vi "LEDComms.vi"() -> (0 "error out":errorcluster)   [LabVIEW 2017]
uses:
  Implements/TypeDefs/IntakeState.ctl
  <vilib>/Rock Robotics/SystemInterfaces/i2clib/i2c_bus.ctl
  Global_Var-RefNum/LEDData.vi
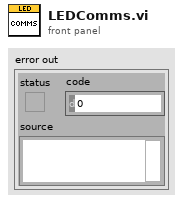
[diagram p1: front panel]
types:
  T1 = typedef "ArmTargetPosition.ctl" = enum16{"Hold", "Switch", "Scale Low", "Scale High", "Climb", "Back Place"}
  T2 = typedef "WPI_DriverStationRobotMode2.ctl" = enum16{"Autonomous Disabled", "Autonomous Enabled", "Teleop Disabled", "Teleop Enabled", "Disconnected", "Finish", "Test Disabled", "Test Enabled", "Emergency Stopped"}
  T3 = typedef "IntakeState.ctl" = enum16{"Stop", "Forward", "Reverse", "Forward Open"}
  T4 = typedef "LEDAutoMode.ctl" = enum16{"Auto Left Switch", "Auto Left Scale", "Auto Center Switch", "Auto Center Scale", "Auto Right Switch", "Auto Right Scale", "Auto Line"}
  T5 = typedef "WPI_I2CDevRef.ctl" = cluster{"DevStatus":errorcluster, "Device Address":u8, "Handle":i32, "I2C Bus":T6}
  T6 = typedef "i2c_bus.ctl" = enum16{"I2C On-Board", "I2C MXP", "Invalid"}
  T7 = typedef "WPI_DriverStationAllianceInfo.ctl" = enum16{"Red", "Blue", "Invalid"}
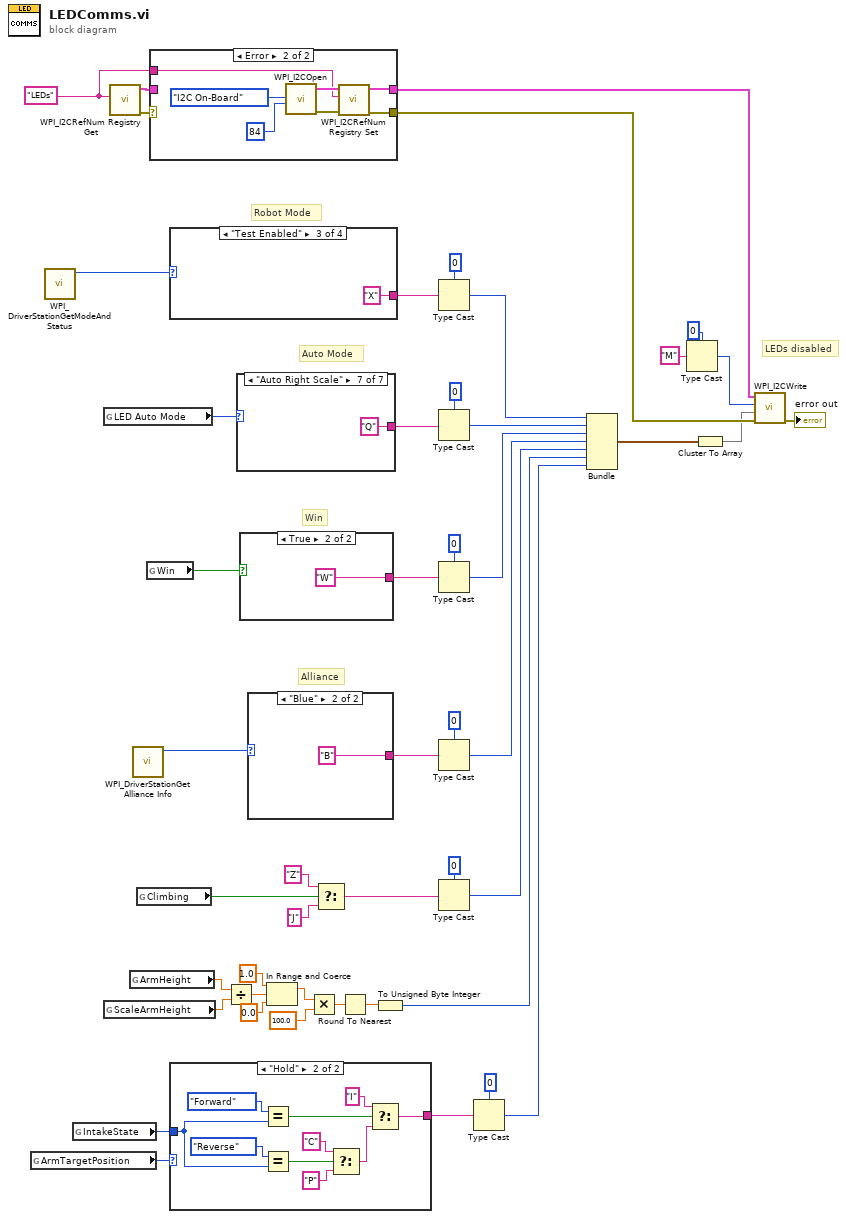
[diagram p0: block diagram]
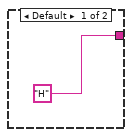
[diagram p2: hidden frame]
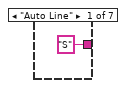
[diagram p4: hidden frame]
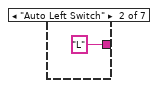
[diagram p5: hidden frame]
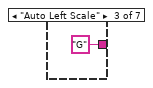
[diagram p6: hidden frame]
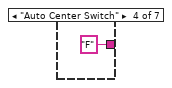
[diagram p7: hidden frame]
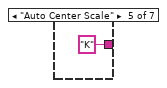
[diagram p8: hidden frame]
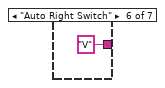
[diagram p9: hidden frame]
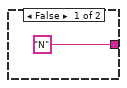
[diagram p10: hidden frame]
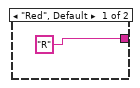
[diagram p11: hidden frame]
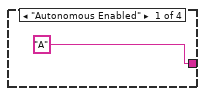
[diagram p12: hidden frame]
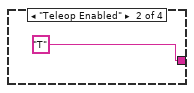
[diagram p13: hidden frame]
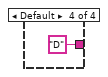
[diagram p14: hidden frame]
diagram:
  w23 = "LEDs" ("refnum name")
  # "LEDs disabled"
  # "Alliance"
  # "Win"
  # "Robot Mode"
  # "Auto Mode"
  n1 = global read "LEDData.vi" "ArmTargetPosition"() -> (w4:T1)
  n2 = call <vilib>:"WPI_DriverStationGetModeAndStatus.vi"() -> ("Robot Mode"=w30:T2)  [unwired: 10 in, 1 out]
  n3 = global read "LEDData.vi" "IntakeState"() -> (w2:T3)
  n4 = global read "LEDData.vi" "LED Auto Mode"() -> (w20:T4)
  n5 = global read "LEDData.vi" "ScaleArmHeight"() -> (w13:dbl)
  n6 = call <vilib>:"WPI_I2CRefNum Registry Get.vi"("refnum name"=w23) -> ("error out"=w21:errorcluster, "I2CDevRef"=w22:T5)  [unwired: 9 in]
  n7 = global read "LEDData.vi" "ArmHeight"() -> (w14:dbl)
  n8 = call <vilib>:"WPI_DriverStationGet Alliance Info.vi"() -> ("Alliance"=w39:T7)  [unwired: 6 in, 5 out]
  n9 = global read "LEDData.vi" "Climbing"() -> (w16:bool)
  n10 = global read "LEDData.vi" "Win"() -> (w19:bool)
  n11 = case shown="Error" w21 {
    selector: w21 -> [w50 _]
    tunnel: [w50 w52] -> w48
    tunnel: [w49 w53] -> w47
    tunnel: w22 -> [w49 _]
    tunnel: w23 -> [_ w51]
    frame No Error {
    }
    frame Error {
      n12 = call <vilib>:"WPI_I2COpen.vi"("Device Address"=u8 84, "I2C Bus"=i2c_bus."I2C On-Board") -> ("error out"=w55:errorcluster, "I2CDevRef"=w54:T5)  [unwired: 8 in]
      n13 = call <vilib>:"WPI_I2CRefNum Registry Set.vi"("error in (no error)"=w55, "refnum name"=w51, "I2CDevRef"=w54) -> ("error out"=w52:errorcluster, "I2CDevRef"=w53:T5)  [unwired: 7 in]
    }
  }
  n14 = case shown="\"Test Enabled\"" w30 {
    tunnel: ["A" "T" "X" "D"] -> w42
    frame "Autonomous Enabled" {
    }
    frame "Teleop Enabled" {
    }
    frame "Test Enabled" {
    }
    frame Default {
    }
  }
  n15 = case shown="\"Hold\"" w4 {
    tunnel: ["H" w63] -> w3
    tunnel: w2 -> [_ w70]
    frame Default {
    }
    frame "Hold" {
      n16 = Equal?(x=IntakeState."Forward", y=w70) -> (x = y?=w64:bool)
      n17 = Equal?(x=IntakeState."Reverse", y=w70) -> (x = y?=w68:bool)
      n18 = Select(t="C", s=w68, f="P") -> (s? t:f=w65:string)
      n19 = Select(t="I", s=w64, f=w65) -> (s? t:f=w63:string)
    }
  }
  n20 = Divide(x=w14, y=w13) -> (x/y=w12:dbl)
  n21 = case shown="\"Auto Right Scale\"" w20 {
    tunnel: ["S" "L" "G" "F" "K" "V" "Q"] -> w24
    frame "Auto Line" {
    }
    frame "Auto Left Switch" {
    }
    frame "Auto Left Scale" {
    }
    frame "Auto Center Switch" {
    }
    frame "Auto Center Scale" {
    }
    frame "Auto Right Switch" {
    }
    frame "Auto Right Scale" {
    }
  }
  n22 = case shown="True" w19 {
    tunnel: ["N" "W"] -> w32
    frame False {
    }
    frame True {
    }
  }
  n23 = case shown="\"Blue\"" w39 {
    tunnel: ["R" "B"] -> w37
    frame "Red", Default {
    }
    frame "Blue" {
    }
  }
  n24 = In Range and Coerce(upper limit=1.0, x=w12, lower limit=0.0) -> (coerced(x)=w9:dbl)  [unwired: 1 out]
  n25 = Multiply(x=w9, y=100.0) -> (x*y=w7:dbl)
  n26 = Select(t="Z", s=w16, f="J") -> (s? t:f=w15:string)
  n27 = Round To Nearest(number=w7) -> (nearest integer value=w6:dbl)
  n28 = To Unsigned Byte Integer(number=w6) -> (unsigned 8bit integer=w5:u8)
  n29 = Type Cast(type=u8 0, x=w42) -> (*(type *) &x=w41:u8)
  n30 = Type Cast(type=u8 0, x=w24) -> (*(type *) &x=w35:u8)
  n31 = Type Cast(type=u8 0, x=w32) -> (*(type *) &x=w33:u8)
  n32 = Type Cast(type=u8 0, x=w37) -> (*(type *) &x=w29:u8)
  n33 = Type Cast(type=u8 0, x=w15) -> (*(type *) &x=w27:u8)
  n34 = Type Cast(type=u8 0, x=w3) -> (*(type *) &x=w25:u8)
  n35 = Bundle(w41, w35, w33, w29, w27, w5, w25) -> (w31:cluster{u8, u8, u8, u8, u8, u8, u8})  [unwired: 1 in]
  n36 = Type Cast(type=u8 0, x="M") -> (*(type *) &x=w44:u8)
  n37 = Cluster To Array(cluster=w31) -> (array=w40:u8[])
  n38 = call <vilib>:"WPI_I2CWrite.vi"("error in (no error)"=w48, "I2CDataToSend"=w40, "I2CRegister"=w44, "I2CDevRef"=w47) -> ("error out"=→"error out":errorcluster)  [unwired: 6 in, 1 out]
